vi "Sensor ID.vi"(8 "error in (no error)":errorcluster, 11 "Scale in":refnum<class "Scale Config.lvclass">) -> (0 "error out":errorcluster, 2 "Sensor ID":string, 3 "Scale out":refnum<class "Scale Config.lvclass">)   [LabVIEW 2020, in "VolatusConfig.lvlib" / "Scale Config.lvclass"]
uses:
  Scale Config.lvclass
  C:/dev/lv20CE/relink/lv-volatus/VolatusConfig/VolatusConfigElement/VolatusConfigElement.lvclass
  VolatusConfigElement/VolatusConfigElement.lvclass/VolatusConfigElement.ctl
  VolatusConfigElement/Element.vi
  Scale Config.lvclass/Scale Config.ctl
  VolatusConfigElement/VolatusConfigElement.lvclass
  lv-cdm/CDM-Config/Config Element/Config Element.lvclass
  C:/dev/lv20CE/relink/lv-volatus/VolatusConfig/Scale/Scale Config.lvclass
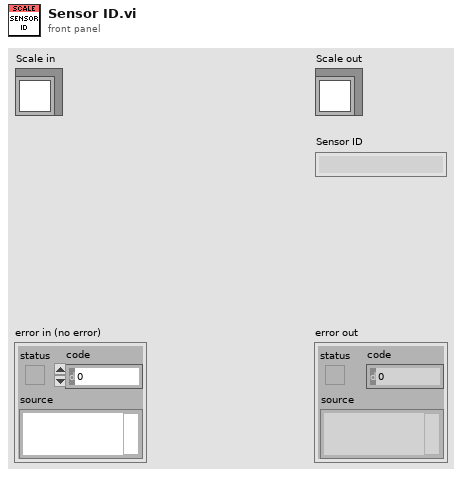
[diagram p1: front panel]
types:
  T1 = typedef "VolatusConfig.lvlib/Scale Type.ctl" = enum16{"None", "Sensor", "Polynomial", "Threshold", "Invert Bool", "Exponential"}
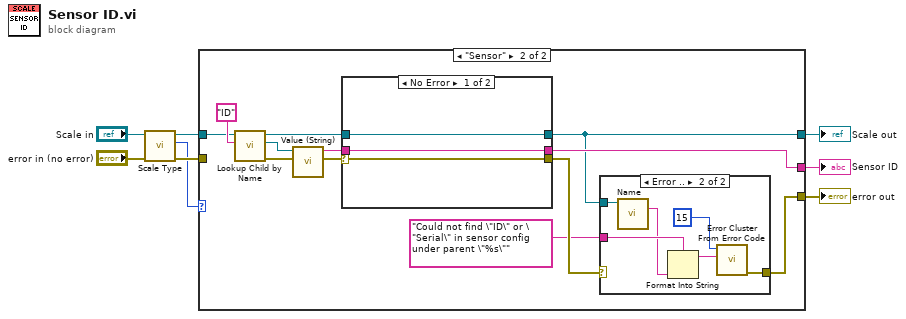
[diagram p0: block diagram]
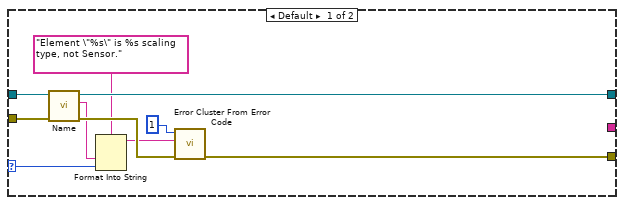
[diagram p2: hidden frame]
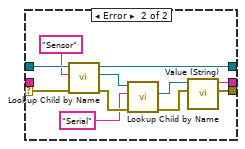
[diagram p3: hidden frame]
diagram:
  n1 = call "Scale Type.vi"("error in (no error)"="error in (no error)", "Scale in"="Scale in") -> ("error out"=w4:errorcluster, "Scale Type"=w1:T1, "Scale out"=w2:refnum<class "Scale Config.lvclass">)  [unwired: 7 in]
  n2 = case shown="\"Sensor\"" w1 {
    selector: w1 -> [w9 _]
    tunnel: [w14 w19] -> w7
    tunnel: [w16 w24] -> w6
    tunnel: [_ w20] -> w5
    tunnel: w4 -> [w13 _]
    tunnel: w2 -> [w17 w25]
    frame Default {
      n3 = call "Name.vi"("error in (no error)"=w13, "VolatusConfigElement in"=w17) -> ("error out"=w18:errorcluster, "Name"=w12:string, "VolatusConfigElement out"=w14:refnum<class "Scale Config.lvclass">)  [unwired: 7 in]
      n4 = Format Into String(format string="Element \"%s\" is %s scaling type, not Sensor.", w12, w9) -> (resulting string=w11:string)  [unwired: 2 in, 1 out]
      n5 = call <vilib>:"Error Cluster From Error Code.vi"("error in (no error)"=w18, "error message (\"\")"=w11, "error code (0)"=1) -> ("error out"=w16:errorcluster)  [unwired: 6 in]
    }
    frame "Sensor" {
      n6 = call "Lookup Child by Name.vi"("Child Name"="ID", "VolatusConfigElement in"=w25) -> ("error out"=w28:errorcluster, "Child"=w27:refnum<class "Config Element.lvclass">, "VolatusConfigElement out"=w23:refnum<class "Scale Config.lvclass">)  [unwired: 6 in, 1 out]
      n7 = call "Value (String).vi"("error in (no error)"=w28, "Config Element in"=w27) -> ("error out"=w21:errorcluster, "String Value"=w22:string)  [unwired: 8 in]
      n8 = case shown="No Error" w21 {
        selector: w21 -> [w33 w37]
        tunnel: w22 -> [w32 _]
        tunnel: w23 -> [w31 w44]
        tunnel: [w32 w42] -> w20
        tunnel: [w31 w41] -> w19
        tunnel: [w33 w40] -> w30
        frame No Error {
        }
        frame Error {
          n9 = call "Lookup Child by Name.vi"("error in (no error)"=w37, "Child Name"="Sensor", "VolatusConfigElement in"=w44) -> ("error out"=w38:errorcluster, "Child"=w39:refnum<class "Config Element.lvclass">, "VolatusConfigElement out"=w41:refnum<class "Scale Config.lvclass">)  [unwired: 5 in, 1 out]
          n10 = call "Lookup Child by Name.vi"("error in (no error)"=w38, "Name"="Serial" ("Child Name"), "Config Element in"=w39) -> ("error out"=w35:errorcluster, "Child"=w36:refnum<class "Config Element.lvclass">)  [unwired: 5 in, 2 out]
          n11 = call "Value (String).vi"("error in (no error)"=w35, "Config Element in"=w36) -> ("error out"=w40:errorcluster, "String Value"=w42:string)  [unwired: 8 in]
        }
      }
      n12 = case shown="Error .." w30 {
        selector: w30 -> [w45 _]
        tunnel: "Could not find \"ID\" or \"Serial\" in sensor config under parent \"%s\"" -> [_ w50]
        tunnel: [w45 w48] -> w24
        tunnel: w19 -> [_ w51]
        frame No Error {
        }
        frame Error {
          n13 = call "Name.vi"("VolatusConfigElement in"=w51) -> ("Name"=w49:string)  [unwired: 8 in, 2 out]
          n14 = Format Into String(format string=w50, w49) -> (resulting string=w46:string)  [unwired: 2 in, 1 out]
          n15 = call <vilib>:"Error Cluster From Error Code.vi"("error message (\"\")"=w46, "error code (0)"=15) -> ("error out"=w48:errorcluster)  [unwired: 7 in]
        }
      }
    }
  }
  "error out" <- w6
  "Scale out" <- w7
  "Sensor ID" <- w5
